vi "Apply Endpoint Configuration.vi"(8 "error in":errorcluster, 9 "endpoint":string, 10 "endpoint configuration in":T1 format="%.0x", 11 "instrument handle in":refnum<k15>) -> (0 "error out":errorcluster, 1 "endpoint addressable?":bool, 2 "endpoint configuration out":T1 format="%.0x", 3 "instrument handle out":refnum<k15>)   [LabVIEW 2020, in "NI-SWITCH Scripting.lvlib"]
uses:
  NI-SWITCH Scripting.lvlib
  <vilib>/NI VeriStand/Custom Device API/Custom Device Item Ref.ctl
  <vilib>/NI VeriStand/Custom Device API/Custom Device API.lvlib
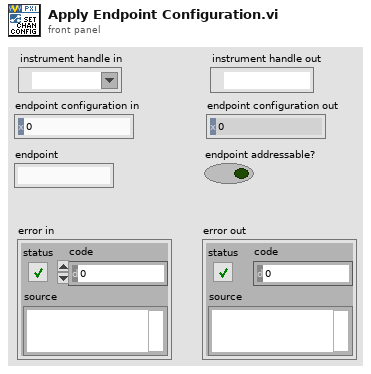
[diagram p1: front panel]
types:
  T1 = typedef "Custom Device API.lvlib/Custom Device Item Ref.ctl" = u64
  T2 = typedef "NI-SWITCH Shared.lvlib/Endpoint Configuration Enum.ctl" = enum16{"Load", "Source", "Configuration"}
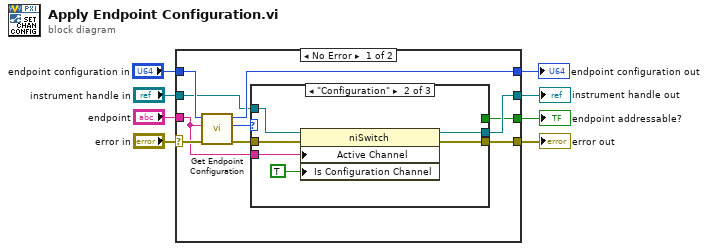
[diagram p0: block diagram]
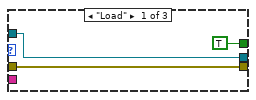
[diagram p2: hidden frame]
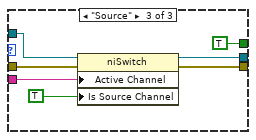
[diagram p3: hidden frame]
diagram:
  n1 = case shown="No Error" "error in" {
    selector: "error in" -> [w14 w37]
    tunnel: [w18 w35] -> w8
    tunnel: [w17 w37] -> w7
    tunnel: [w15 w36] -> w2
    tunnel: "endpoint configuration in" -> [w13 w35]
    tunnel: "endpoint" -> [w12 _]
    tunnel: [w10 _] -> w3
    tunnel: "instrument handle in" -> [w9 w36]
    frame No Error {
      n2 = call "Get Endpoint Configuration.vi"("error in"=w14, "endpoint"=w12, "endpoint configuration in"=w13) -> ("error out"=w16:errorcluster, "configuration"=w11:T2, "endpoint configuration out"=w18:T1)  [unwired: 6 in]
      n3 = case shown="\"Configuration\"" w11 {
        tunnel: w9 -> [w20 w26 w34]
        tunnel: w12 -> [_ w27 w32]
        tunnel: [TRUE _ TRUE] -> w10
        tunnel: [w20 w24 w30] -> w15
        tunnel: w16 -> [w19 w23 w28]
        tunnel: [w19 w22 w29] -> w17
        frame "Load" {
        }
        frame "Configuration" {
          n4 = property class="niSwitch"(reference=w26, error in=w23, "Active Channel"=w27, "Is Configuration Channel"=TRUE ("Channel Configuration:Is Configuration Channel")) -> (reference out=w24:refnum<k15>, error out=w22:errorcluster)
        }
        frame "Source" {
          n5 = property class="niSwitch"(reference=w34, error in=w28, "Active Channel"=w32, "Is Source Channel"=TRUE ("Channel Configuration:Is Source Channel")) -> (reference out=w30:refnum<k15>, error out=w29:errorcluster)
        }
      }
    }
    frame Error {
    }
  }
  "endpoint configuration out" <- w8
  "error out" <- w7
  "endpoint addressable?" <- w3
  "instrument handle out" <- w2
